vi "Get Running Entry.vi"(7 "Time Entry Store in":refnum<class "Time Entry Store-INI.lvclass">, 8 "error in (no error)":errorcluster) -> (0 "error out":errorcluster, 2 "found?":bool, 3 "Time Entry":T1, 5 "Time Entry Store out":refnum<class "Time Entry Store-INI.lvclass">)   [LabVIEW 2024, in "Time Entry Store-INI.lvclass"]
doc: "Returns the running time entry - the one whose End Time is 0 - from the month file of the current UTC month or the month before. found? is FALSE when nothing is running. If several are running, the one that started last is returned.\n\nGenerated by: Claude"
uses:
  Time Entry Store-INI.lvclass
  Rows/Time Entry.ctl
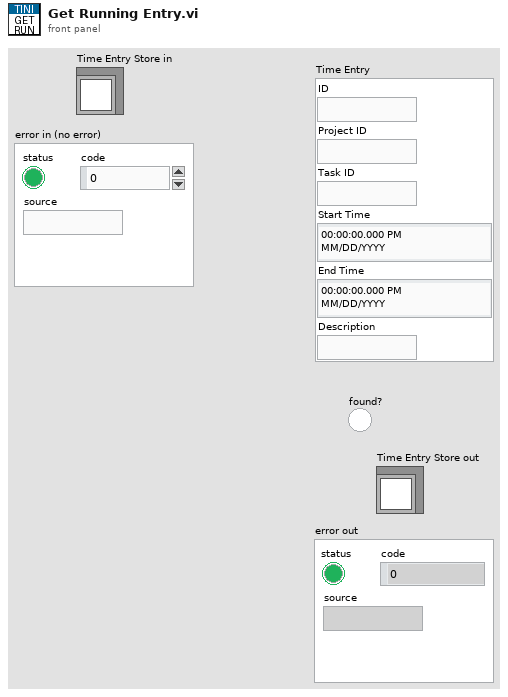
[diagram p1: front panel]
types:
  T1 = typedef "Time Entry.ctl" = cluster{"ID":string, "Project ID":string, "Task ID":string, "Start Time":timestamp, "End Time":timestamp, "Description":string}
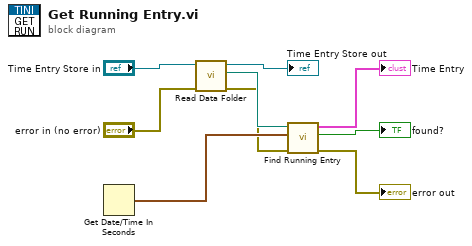
[diagram p0: block diagram]
diagram:
  n1 = Get Date/Time In Seconds() -> (seconds since 1Jan1904=w6:timestamp)
  n2 = call-dynamic "Read Data Folder.vi"("error in (no error)"="error in (no error)", "Time Entry Store-INI in"="Time Entry Store in") -> ("error out"=w3:errorcluster, "Data Folder"=w5:path, "Time Entry Store-INI out"=→"Time Entry Store out":refnum<class "Time Entry Store-INI.lvclass">)  [unwired: 7 in]
  n3 = call "Find Running Entry.vi"("error in (no error)"=w3, "Now"=w6, "Data Folder"=w5) -> ("error out"=→"error out":errorcluster, "found?"=→"found?":bool, "Time Entry"=→"Time Entry":T1)  [unwired: 6 in]
